vi "Untitled 3.vi"() -> ()   [LabVIEW 2018]
panel:
  out "Numeric 3":dbl
  in  "Numeric 2":dbl
  in  "Numeric":dbl
  # "f=(1.8*C)+32"
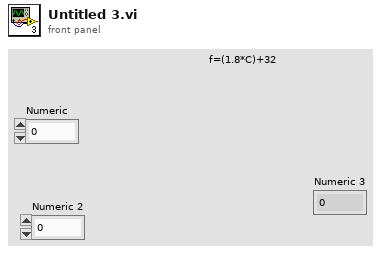
[diagram p1: front panel]
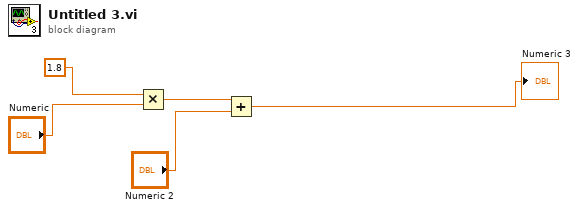
[diagram p0: block diagram]
diagram:
  n1 = Multiply(x=1.8, y="Numeric") -> (x*y=w3:dbl)
  n2 = Add(x=w3, y="Numeric 2") -> (x+y=→"Numeric 3":dbl)
